vi "VIH HelpGen - Write HTML File - Menu.vi"(6 "Owning Palette":cluster{"Name":string, "HTML Path":path}, 7 "Items":T2, 8 "error in":errorcluster, 9 "HTML Path":path, 10 "Menu Path":path, 11 "Project Tree":T1) -> (0 "error out":errorcluster, 3 "dup Project Tree":T1)   [LabVIEW 2014]
doc: "::: VI Helpeks :::\nCopyright (c) 2000-2026 Konstantin Shifershteyn. All rights reserved."
uses:
  _VIH Project Manager.llb/VIH Project Tree Typedef - Tree Refnum.ctl
  VIH HelpGen Typedef - Enum - Default,Enable,Disable.ctl
panel:
  # "VI Helpeks\nCopyright (c) 2012-2026 Konstantin Shifershteyn"
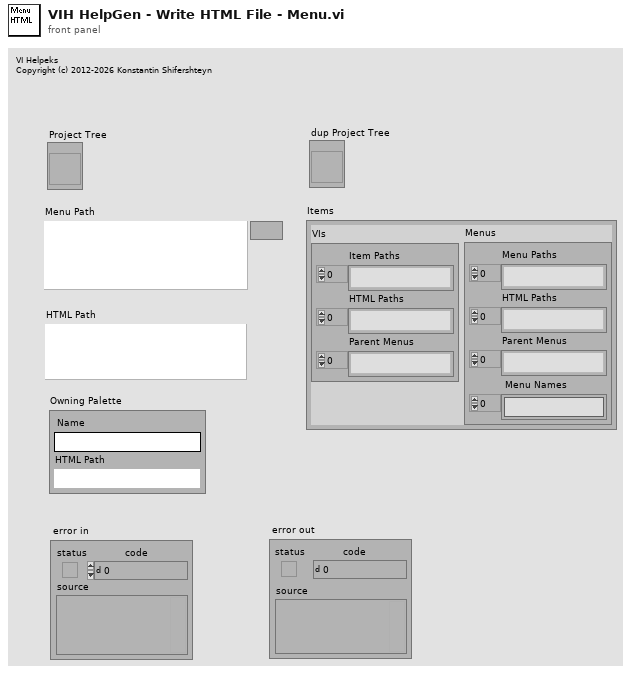
[diagram p1: front panel]
types:
  T1 = typedef "VIH Project Tree Typedef - Tree Refnum.ctl" = refnum<vi>
  T2 = cluster{"VIs":cluster{"Item Paths":path[], "HTML Paths":path[], "Parent Menus":path[]}, "Menus":cluster{"Menu Paths":path[], "HTML Paths":path[], "Parent Menus":path[], " Menu Names":string[]}}
  T3 = typedef "VIH HelpGen Typedef - Enum - Default,Enable,Disable.ctl" = enum16{"Default", "Enable", "Disable"}
  T4 = typedef "VIH HelpGen Typedef - Cluster - File Rule.ctl" = cluster{"OutName":string, "BuildHelp":T3, "Source Paths":T5, "Target Paths":T6, "DscrMode":T7, "Description":string, "Control Rules":T8[], "Flags":T10, "Ctl_DscrMode":T7, "Ctl_ClustMembers":T3, "Ctl_EnumValues":T3, "MenuItemIcons":T3, "%Comments":string, "DetailsMode":T7, "DetailsText":string, "ProductInfoMode":T3, "ProductInfoText":string}
  T5 = typedef "VIH HelpGen Typedef - Cluster - File Rule - Source Paths.ctl" = cluster{"CSS Files":path[], "JS Files":path[], "Html Template":path}
  T6 = typedef "VIH HelpGen Typedef - Cluster - File Rule - Target Paths.ctl" = cluster{"HTML Dir":path, "Image Dir":path, "CSS Dir":path, "JS Dir":path}
  T7 = typedef "VIH HelpGen Typedef - Enum - Description Mode.ctl" = enum16{"Default", "Description", "Description1", "Description2", "Custom", "None"}
  T8 = typedef "VIH HelpGen Typedef - Cluster - Control Rule.ctl" = cluster{"CtrlID":string, "CustomRule":bool, "DscrMode":T7, "Description":string, "ClusterMembers":T3, "EnumValues":T3, "EnumValDscr":T9[], "CustomName":string}
  T9 = typedef "VIH HelpGen Typedef - Cluster - Enum Value Info.ctl" = cluster{"Value":ext, "String":string, "Description":string}
  T10 = typedef "VIH HelpGen Typedef - Cluster - Group Rule - Flags.ctl" = cluster{"Override CSS Files":bool, "Override JS Files":bool, "Override Ctl Rules":bool}
  T11 = cluster{"ProductInfoMode":T3, "ProductInfoText":string}
  T12 = typedef "VIH HelpGen Typedef - Table Templates Cluster - Menu Help.ctl" = cluster{"Objects":string, "Sub-palettes":string}
  T13 = cluster{"directory path out":path, "directory path out":path, "name":string}
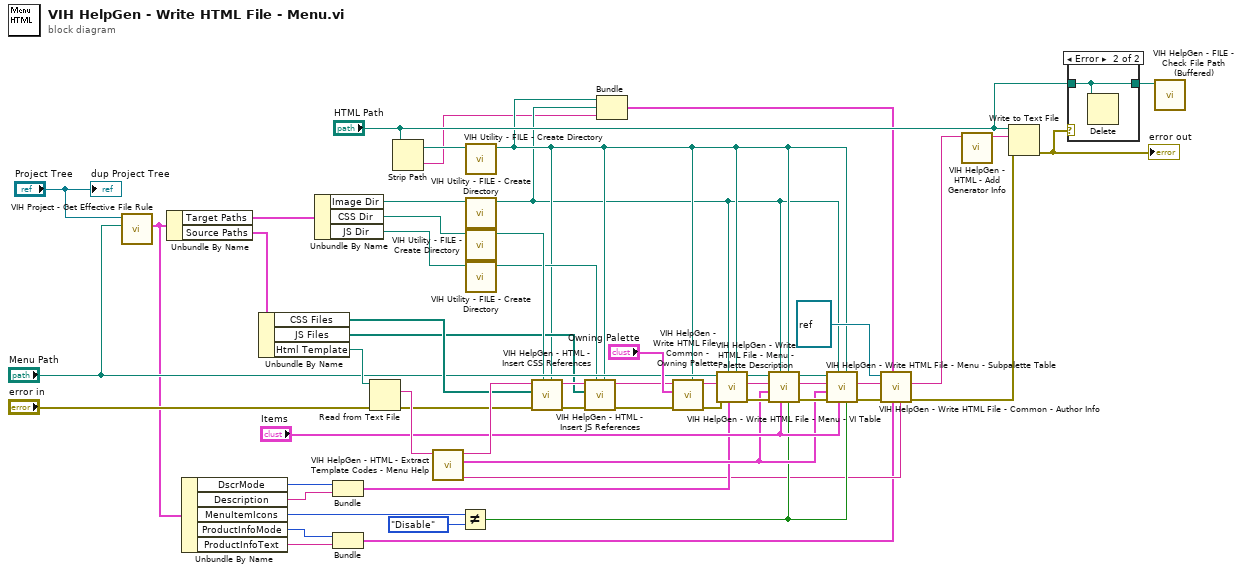
[diagram p0: block diagram]
diagram:
  n1 = call "VIH Project - Get Effective File Rule.vi"("File Path"="Menu Path", "Project Tree"="Project Tree") -> ("Effective File Rule"=w29:T4)  [unwired: 6 in, 3 out]
  n2 = Unbundle By Name(w29) -> ("Target Paths"=w54:T6, "Source Paths"=w53:T5)
  n3 = Unbundle By Name(w29) -> ("DscrMode"=w30:T7, "Description"=w31:string, "MenuItemIcons"=w20:T3, "ProductInfoMode"=w7:T3, "ProductInfoText"=w8:string)
  n4 = Unbundle By Name(w53) -> ("CSS Files"=w52:path[], "JS Files"=w21:path[], "Html Template"=w51:path)
  n5 = Unbundle By Name(w54) -> ("Image Dir"=w32:path, "CSS Dir"=w34:path, "JS Dir"=w23:path)
  n6 = Bundle("DscrMode"=w30, "Description"=w31) -> (w28:cluster{"DscrMode":T7, "Description":string})  [unwired: 1 in]
  n7 = Bundle("ProductInfoMode"=w7, "ProductInfoText"=w8) -> (w6:T11)  [unwired: 1 in]
  n8 = Read from Text File(file (use dialog)=w51, error in="error in") -> (text=w56:string, error out=w50:errorcluster)  [unwired: 2 in, 2 out]
  n9 = Strip Path(path="HTML Path") -> (stripped path=w35:path, name=w2:string)
  n10 = call "VIH HelpGen - HTML - Extract Template Codes - Menu Help.vi"("HTML in"=w56) -> ("ProductInfo Template"=w9:string, "Table Templates"=w41:T12, "HTML out"=w55:string)  [unwired: 8 in]
  n11 = Not Equal?(x=w20, y=VIH_HelpGen_Typedef_-_Enum_-_Default,Enable,Disable."Disable") -> (x != y?=w18:bool)
  n12 = call "VIH Utility - FILE - Create Directory.vi"("directory path"=w35) -> ("directory path out"=w4:path)  [unwired: 6 in, 2 out]
  n13 = call "VIH Utility - FILE - Create Directory.vi"("directory path"=w32) -> ("directory path out"=w3:path)  [unwired: 6 in, 2 out]
  n14 = call "VIH Utility - FILE - Create Directory.vi"("directory path"=w34) -> ("directory path out"=w33:path)  [unwired: 6 in, 2 out]
  n15 = call "VIH Utility - FILE - Create Directory.vi"("directory path"=w23) -> ("directory path out"=w22:path)  [unwired: 6 in, 2 out]
  n16 = call "VIH HelpGen - HTML - Insert CSS References.vi"("HTML Folder"=w4, "CSS Folder"=w33, "error in"=w50, "CSS files"=w52, "HTML in"=w55) -> ("error out"=w26:errorcluster, "HTML out"=w27:string)  [unwired: 5 in]
  n17 = call "VIH HelpGen - HTML - Insert JS References.vi"("HTML Folder"=w4, "JSS Folder"=w22, "error in"=w26, "JS files"=w21, "HTML in"=w27) -> ("error out"=w25:errorcluster, "HTML out"=w24:string)  [unwired: 5 in]
  n18 = Bundle("directory path out"=w4, "directory path out"=w3, "name"=w2) -> (w1:T13)  [unwired: 1 in]
  n19 = call "VIH HelpGen - Write HTML File - Common - Owning Palette.vi"("HTML Folder"=w4, "error in"=w25, "Owning Palette"="Owning Palette", "HTML in"=w24) -> ("error out"=w38:errorcluster, "HTML out"=w39:string)  [unwired: 6 in]
  n20 = call "VIH HelpGen - Write HTML File - Menu - Palette Description.vi"("HTML Folder"=w4, "Description Params"=w28, "Image Folder"=w3, "error in"=w38, "HTML in"=w39, "Menu Path"="Menu Path") -> ("error out"=w47:errorcluster, "HTML out"=w48:string, "dup Menu Path"=w46:path)  [unwired: 3 in]
  n21 = call "VIH HelpGen - Write HTML File - Menu - VI Table.vi"("Show Item Icons"=w18, "HTML Folder"=w4, "Items"="Items", "Image Folder"=w3, "error in"=w47, "Table Templates"=w41, "HTML in"=w48, "Menu Path"=w46) -> ("error out"=w43:errorcluster, "HTML out"=w44:string, "dup Menu Path"=w45:path)  [unwired: 1 in]
  n22 = call "VIH HelpGen - Write HTML File - Menu - Subpalette Table.vi"("Show Item Icons"=w18, "HTML Folder"=w4, "Items"="Items", "Image Folder"=w3, "error in"=w43, "Table Templates"=w41, "HTML in"=w44, "Menu Path"=w45) -> ("error out"=w11:errorcluster, "HTML out"=w13:string)  [unwired: 2 in]
  n23 = call "VIH HelpGen - Write HTML File - Common - Author Info.vi"("Product Info Template"=w9, "Product Info"=w6, "Save params"=w1, "error in"=w11, "HTML in"=w13, "VI Reference"=refnum<vi> refnum) -> ("error out"=w10:errorcluster, "HTML out"=w12:string)  [unwired: 3 in, 1 out]
  n24 = call "VIH HelpGen - HTML - Add Generator Info.vi"("HTML in"=w12) -> ("HTML out"=w14:string)  [unwired: 10 in]
  n25 = Write to Text File(file (use dialog)="HTML Path", text=w14, error in=w10) -> (error out=w15:errorcluster)  [unwired: 1 in, 2 out]
  "error out" <- w15
  n26 = case shown="Error" w15 {
    tunnel: "HTML Path" -> [w57 w58]
    tunnel: [w57 w58] -> w17
    frame No Error {
    }
    frame Error {
      n27 = Delete(path (use dialog)=w58) -> ()  [unwired: 4 in, 3 out]
    }
  }
  n28 = call "VIH HelpGen - FILE - Check File Path (Buffered).vi"("File Path"=w17) -> ()  [unwired: 9 in, 2 out]
  "dup Project Tree" <- "Project Tree"
